vi "Write Stream State.vi"(7 "last probe":u32, 8 "error in":errorcluster, 9 "last progress":dbl=nan, 10 "cancelled?":bool, 11 "stream key":string) -> (0 "error out":errorcluster)   [LabVIEW 2020, in "MCP Server.lvlib"]
doc: "Stores the state of the streamed tools/call that is running in Stream State.vi: {\"key\",\"last\",\"cancelled\",\"probe\"}, read back by Read Stream State.vi. Used by Report Progress.vi and Cancel Requested.vi.\n\nDoes nothing when stream key is empty (the request is not streamed). last progress NaN is stored as null (no progress sent yet).\n\nRuns regardless of error in, which is passed through unchanged."
uses:
  MCP Server.lvlib
  7a59f17e-f710-4a5b-b28f-4f61cf705398.vi
  1aeccbbb-391a-4a9e-aec3-91f873d322f3.vi
  <vilib>/JDP Science/JSONtext/Variant to JSON Text.vi
  <vilib>/JDP Science/JSONtext/LVClass Serializer/JSONtext LVClass Serializer.lvclass
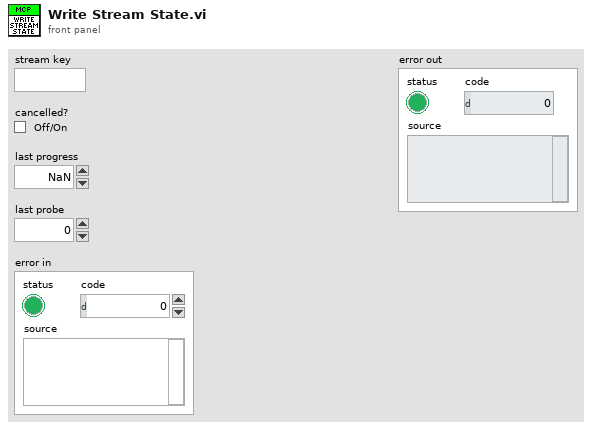
[diagram p1: front panel]
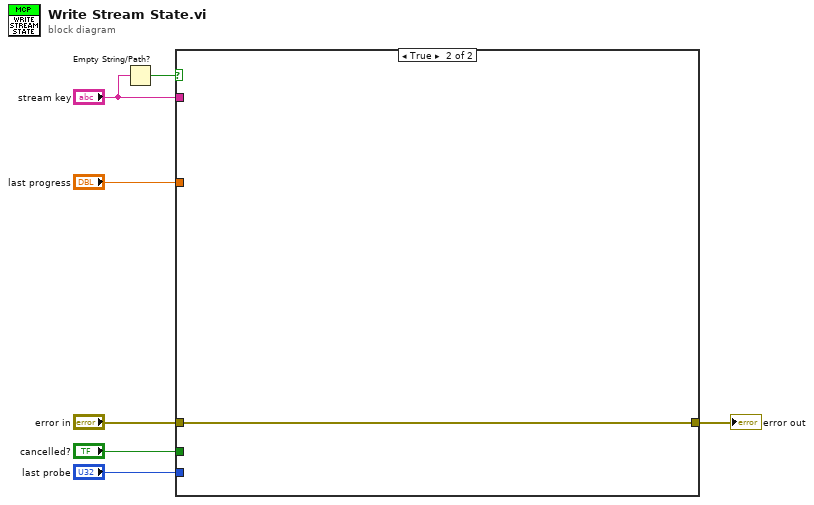
[diagram p0: block diagram]
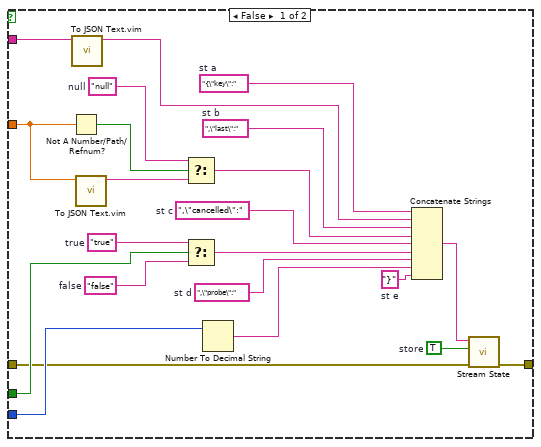
[diagram p2: hidden frame]
diagram:
  n1 = Empty String/Path?(string/path="stream key") -> (empty?=w2:bool)
  n2 = case shown="True" w2 {
    tunnel: "stream key" -> [w29 _]
    tunnel: "cancelled?" -> [w23 _]
    tunnel: "last progress" -> [w28 _]
    tunnel: "last probe" -> [w21 _]
    tunnel: "error in" -> [w9 w30]
    tunnel: [w8 w30] -> w1
    frame False {
      w10 = TRUE  # store
      w22 = "false"  # false
      w24 = "true"  # true
      w27 = "null"  # null
      w12 = "}"  # st e
      w14 = ",\"probe\":"  # st d
      w16 = ",\"cancelled\":"  # st c
      w18 = ",\"last\":"  # st b
      w20 = "{\"key\":"  # st a
      n3 = Not A Number/Path/Refnum?(number/path/refnum=w28) -> (NaN/Path/Refnum?=w26:bool)
      n4 = call "To JSON Text.vim"("Anything"=w29) -> ("<JSON>"=w19:string)  [unwired: 9 in, 1 out]
      n5 = call "To JSON Text.vim"("Anything"=w28) -> ("<JSON>"=w25:string)  [unwired: 9 in, 1 out]
      n6 = Select(t=w27, s=w26, f=w25) -> (s? t:f=w17:string)
      n7 = Select(t=w24, s=w23, f=w22) -> (s? t:f=w15:string)
      n8 = Number To Decimal String(number=w21) -> (decimal integer string=w13:string)  [unwired: 1 in]
      n9 = Concatenate Strings(w20, w19, w18, w17, w16, w15, w14, w13, w12) -> (w11:string)
      n10 = call "Stream State.vi"("error in"=w9, "set?"=w10, "state in"=w11) -> ("error out"=w8:errorcluster)  [unwired: 7 in, 1 out]
    }
    frame True {
    }
  }
  "error out" <- w1
